vi "Set Max File Size.vi"(7 "nSplitTime":u32, 8 "error in (no error)":errorcluster caption="错误输入（无错误）", 9 "nFileSize":u32, 10 "nCutMode":i32, 11 "nRunMode":i32) -> (0 "error out":errorcluster caption="错误输出", 3 "function return":i32)   [LabVIEW 2017, in "smncsftmt.lvlib"]
doc: "__declspec(dllexport) int SetMaxFileSize(int nRunMode, int nCutMode, unsigned int nFileSize, unsigned int nSplitTime);"
uses:
  smncsftmt.lvlib
  smncsftmt.dll
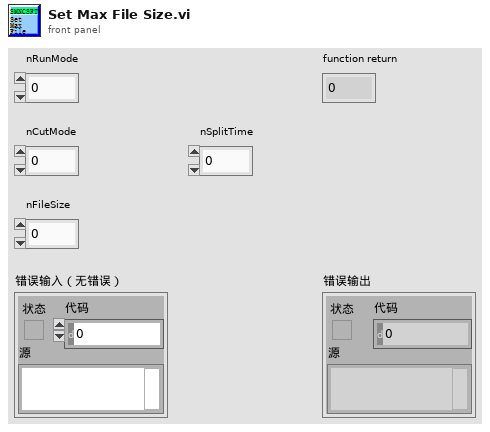
[diagram p1: front panel]
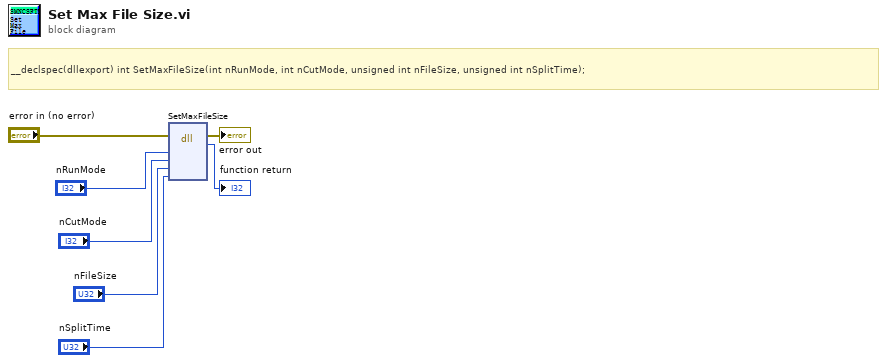
[diagram p0: block diagram]
diagram:
  # "__declspec(dllexport) int SetMaxFileSize(int nRunMode, int nCutMode, unsigned int nFileSize, unsigned int nSplitTime);"
  n1 = dll-call lib="PTH2oabs CUsersaDesktop\nLABVIEW范例National InstrumentsLabVIEW 2017user.lib\tsmncsftmtsmncsftmt.*" fn="SetMaxFileSize"(error in="error in (no error)", "nRunMode"="nRunMode", "nCutMode"="nCutMode", "nFileSize"="nFileSize", "nSplitTime"="nSplitTime") -> (error out=→"error out":errorcluster, →"function return":i32)  [unwired: 6 in, 1 out]
